vi "Update Configuration.vi"(8 "error in (no error)":errorcluster, 11 "CIFPlugin in":refnum<class "CAN_Writer_CANsub_Plugin.lvclass">) -> (0 "error out":errorcluster, 3 "CIFPlugin out":refnum<class "CAN_Writer_CANsub_Plugin.lvclass">)   [LabVIEW 2021, in "CAN_Writer_CANsub_Plugin.lvclass"]
uses:
  CAN_Writer_CANsub_Plugin.lvclass
  CAN_Writer_CANsub_Plugin.lvclass/CAN_Writer_CANsub_Plugin.ctl
  <vilib>/CIF Foundation/CIF Core/CIFCore/Class/CIFCorePlugin.lvclass
  C:/Program Files/National Instruments/LabVIEW 2021/vi.lib/CIF Foundation/CIF Core/CIFCore/Class/CIFCorePlugin.lvclass
  <vilib>/CIF Foundation/CIF XNET CAN RW/XNET CAN RW.lvclass
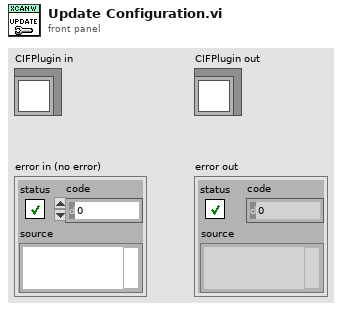
[diagram p1: front panel]
types:
  T1 = typedef "CAN_Writer_CANsub_Common.lvlib/Configuration.ctl" = cluster{"Common":T2, "TX Interface":string, "Port Configuration":T4, "Filter":T7, "Wake Offset (us)":i64, "One Shot":bool}
  T2 = typedef "CIFCoreCommon.lvlib/Common Plugin Configuration.ctl" = cluster{"Period (s)":dbl, "Offset (us)":i32, "Priority":i32, "Processor":i32, "External Clock":T3}
  T3 = typedef "CIFCoreCommon.lvlib/External Clock Config.ctl" = cluster{"ClockID":u8, "Clock Name":string, "Publish Clock":bool, "Convert Data Timestamps":bool, "Plugin Timing Source":bool}
  T4 = typedef "CAN_RW_CORE.lvclass/CAN Port Configuration.ctl" = cluster{"Mode":T5, "Baud Rate":u64, "Temination On":bool, "Subordinate":bool, "Echo TX":bool, "FD Config":T6}
  T5 = typedef "CAN_RW_CORE.lvclass/CAN Mode.ctl" = enum16{"CAN 2.0", "CAN FD"}
  T6 = typedef "CAN_RW_CORE.lvclass/FD Config.ctl" = cluster{"FD Baud Rate":u64, "ISO Mode":bool, "BRS Enabled":bool}
  T7 = typedef "CAN_RW_CORE.lvclass/CAN Filter.ctl" = cluster{"Allow List (ID)":u32[], "Deny List (ID)":u32[]}
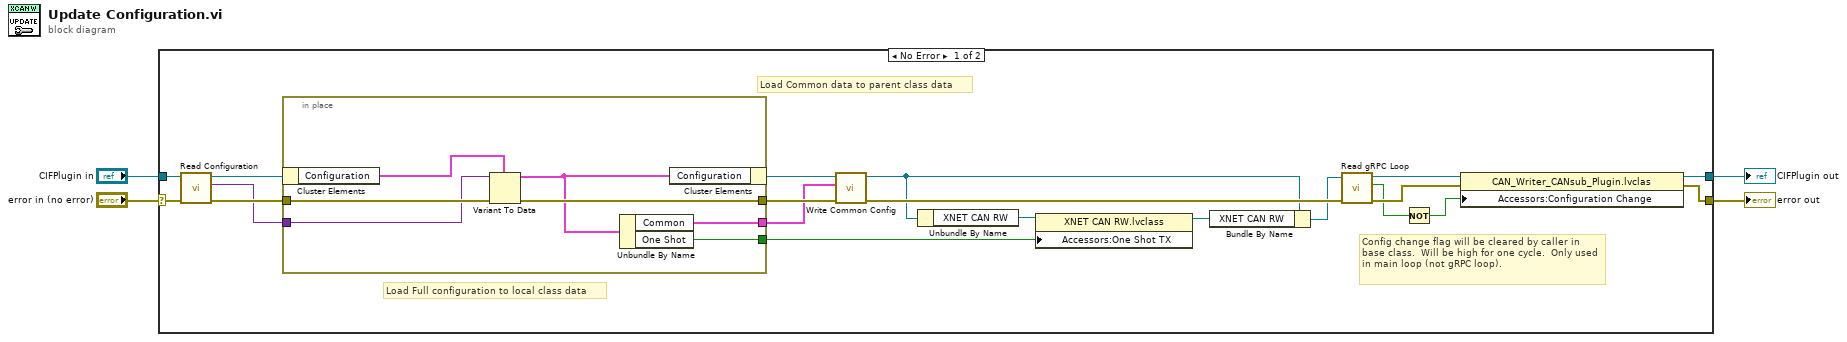
[diagram p0: block diagram]
diagram:
  n1 = case shown="No Error" "error in (no error)" {
    selector: "error in (no error)" -> [w20 w32]
    tunnel: "CIFPlugin in" -> [w21 w33]
    tunnel: [w16 w33] -> w1
    tunnel: [w15 w32] -> w3
    frame No Error {
      # "Config change flag will be cleared by caller in base class.  Will be high for one cycle.  Only used in main loop (not gRPC loop)."
      # "Load Common data to parent class data"
      # "Load Full configuration to local class data"
      n2 = call <vilib>:"Read Configuration.vi"("error in"=w20, "CIFCorePlugin in"=w21) -> ("error out"=w19:errorcluster, "Configuration Data"=w18:variant, "CIFCorePlugin in"=w17:refnum<class "CAN_Writer_CANsub_Plugin.lvclass">)  [unwired: 7 in]
      n3 = in-place {
        in-place-border: [w31] -> w24
        in-place-border: w19 -> [w30]
        in-place-border: w18 -> [w29]
        in-place-border: [w27] -> w23
        in-place-border: [w25] -> w8
        n4 = in-place-cluster #1(w17) -> ("Configuration"=w28:T1)
        n5 = Variant To Data(error in=w30, type=w28, Variant=w29) -> (data=w26:T1, error out=w31:errorcluster)
        n6 = Unbundle By Name(w26) -> ("Common"=w27:T2, "One Shot"=w25:bool)
        n7 = in-place-cluster #1("Configuration"=w26) -> (w22:refnum<class "CAN_Writer_CANsub_Plugin.lvclass">)
      }
      n8 = call <vilib>:"Write Common Config.vi"("error in (no error)"=w24, "Common"=w23, "CIFTemplateNode in"=w22) -> ("error out"=w14:errorcluster, "CIFTemplateNode in"=w7:refnum<class "CAN_Writer_CANsub_Plugin.lvclass">)  [unwired: 7 in]
      n9 = Unbundle By Name(w7) -> ("XNET CAN RW"=w9:refnum<class "XNET CAN RW.lvclass">)
      n10 = property class="XNET CAN RW.lvclass"(reference=w9, "Accessors:One Shot TX"=w8) -> (reference out=w6:refnum<class "XNET CAN RW.lvclass">)  [unwired: 1 in, 1 out]
      n11 = Bundle By Name(cluster=w7, "XNET CAN RW"=w6) -> (w5:refnum<class "CAN_Writer_CANsub_Plugin.lvclass">)
      n12 = call <vilib>:"Read gRPC Loop.vi"("error in (no error)"=w14, "CIFCorePlugin in"=w5) -> ("error out"=w12:errorcluster, "gRPC Loop"=w10:bool, "CIFCorePlugin in"=w13:refnum<class "CAN_Writer_CANsub_Plugin.lvclass">)  [unwired: 7 in]
      n13 = Not(x=w10) -> (.not. x?=w11:bool)
      n14 = property class="CAN_Writer_CANsub_Plugin.lvclas"(reference=w13, error in=w12, "Accessors:Configuration Change"=w11) -> (reference out=w16:refnum<class "CAN_Writer_CANsub_Plugin.lvclass">, error out=w15:errorcluster)
    }
    frame Error {
    }
  }
  "error out" <- w3
  "CIFPlugin out" <- w1
